vi "UMLEditor SyncCodeFromUml.vi"(7 "Don't Prompt (False)":bool, 8 "error in":errorcluster, 10 "graph":refnum<class "Graph.lvclass">, 11 "selectedNode":refnum<class "AbstractNode.lvclass">) -> (0 "error out":errorcluster)   [LabVIEW 2020]
uses:
  <resource>/Framework/Providers/Open_GDS/UML/AbstractNode_class/AbstractNode.lvclass
  <resource>/Framework/Providers/Open_GDS/UML/Graph_class/Graph.lvclass
  <resource>/Framework/Providers/Open_GDS/UML/ClassNode_class/ExternalSetTypes.ctl
  <resource>/Framework/Providers/Open_GDS/UML/ClassNode_class/ClassNode.lvclass
  C:/Program Files (x86)/National Instruments/LabVIEW 2020/resource/Framework/Providers/Open_GDS/UML/AbstractNode_class/AbstractNode.lvclass
  <resource>/Framework/Providers/Open_GDS/ClassProviders/Common/CommonVIs/CommonVIs_ClassNamePathType.ctl
  <resource>/Framework/Providers/Open_GDS/UML/ClassRelationshipEdge_class/ClassRelationshipEdge.lvclass
  <resource>/Framework/Providers/Open_GDS/UML/AbstractEdge_class/AbstractEdge.lvclass
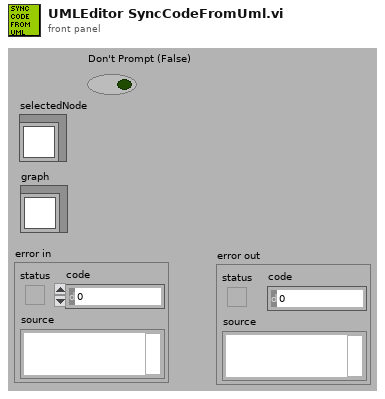
[diagram p1: front panel]
types:
  T1 = typedef "ClassNode.lvclass/ExternalSetTypes.ctl" = enum16{"Name", "Attributes", "Methods", "Position", "ShowMethods", "ShowAttributes", "ClassPath"}
  T2 = typedef "CommonVIs_ClassNamePathType.ctl" = cluster{"ClassNamn":string, "ClassPath":path, "InterfaceClass":bool}
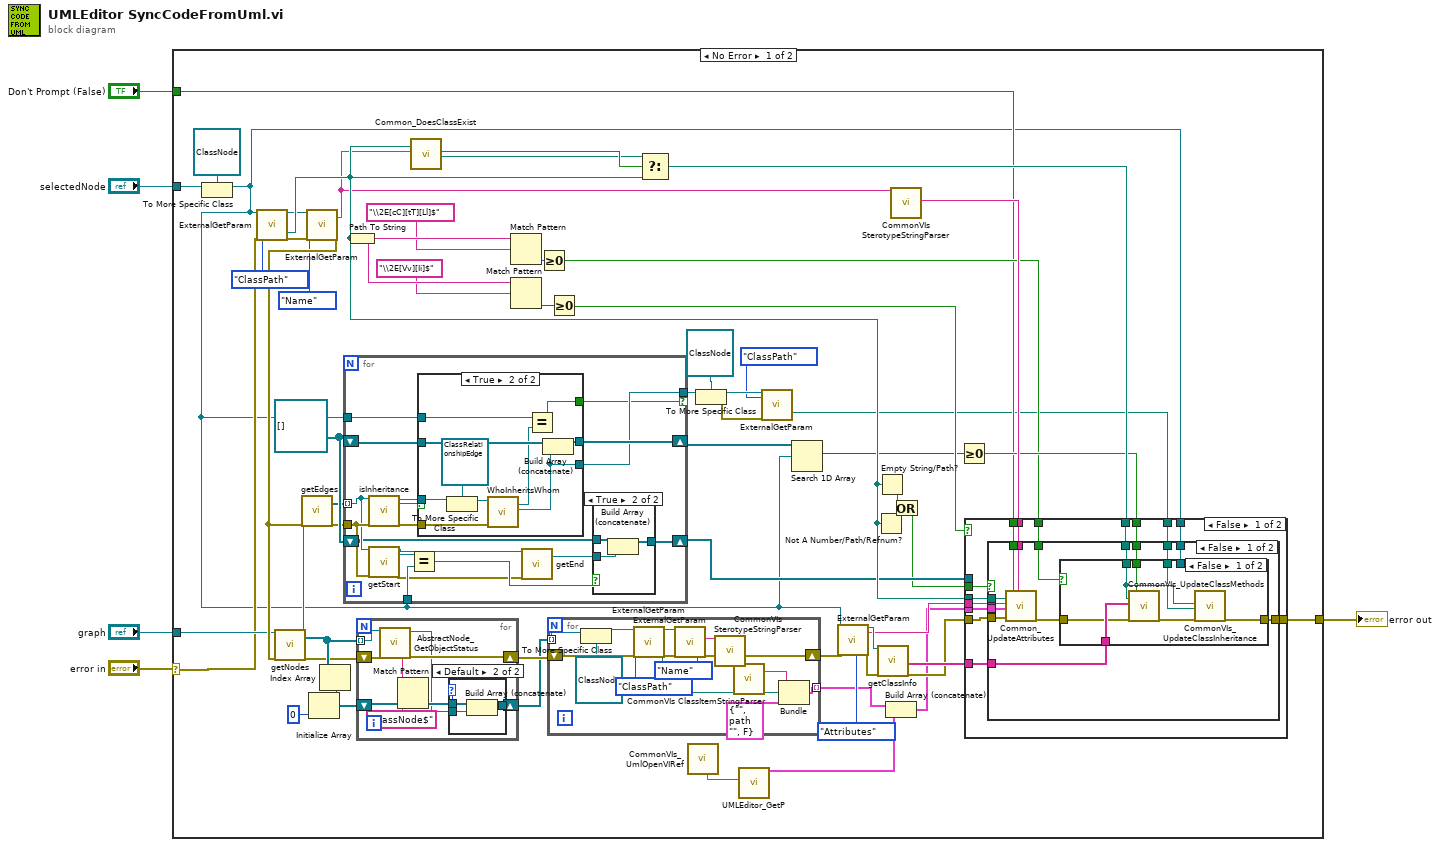
[diagram p0: block diagram]
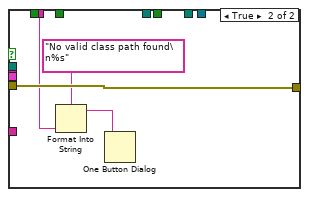
[diagram p3: hidden frame]
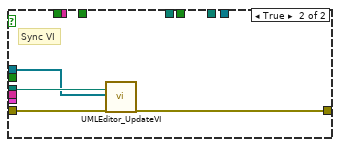
[diagram p4: hidden frame]
diagram:
  n1 = case shown="No Error" "error in" {
    selector: "error in" -> [w13 w171]
    tunnel: [w43 w171] -> w5
    tunnel: "graph" -> [w27 _]
    tunnel: "Don't Prompt (False)" -> [w20 _]
    tunnel: "selectedNode" -> [w14 _]
    frame No Error {
      w63 = refnum<class "AbstractNode.lvclass">[] []
      n2 = To More Specific Class(target class=refnum<class "ClassNode.lvclass"> refnum ("reference"), reference=w14) -> (specific class reference=w12:refnum<class "ClassNode.lvclass">)  [unwired: 1 in, 1 out]
      n3 = call <resource>:"ExternalGetParam.vi"("reference"=w12, "setParameter"=ExternalSetTypes."ClassPath", "error in (no error)"=w13) -> ("reference out"=w44:refnum<class "ClassNode.lvclass">, "Path"=w65:path, "error out"=w45:errorcluster)  [unwired: 14 out]
      n4 = call <resource>:"ExternalGetParam.vi"("reference"=w44, "setParameter"=ExternalSetTypes."Name", "error in (no error)"=w45) -> ("string"=w55:string, "error out"=w47:errorcluster)  [unwired: 15 out]
      n5 = call-dynamic "getNodes.vi"("reference"=w27, "error in (no error)"=w47) -> ("reference out"=w48:refnum<class "Graph.lvclass">, "nodes"=w26:refnum<class "AbstractNode.lvclass">[], "error out"=w25:errorcluster)  [unwired: 15 in]
      n6 = call-dynamic "getEdges.vi"("reference"=w48, "error in (no error)"=w47) -> ("edges"=w50:refnum<class "AbstractEdge.lvclass">[], "error out"=w49:errorcluster)  [unwired: 15 in, 1 out]
      n7 = Index Array(array=w26) -> (element=w22:refnum<class "AbstractNode.lvclass">)  [unwired: 1 in]
      n8 = Initialize Array(w22, 0 ("dimension size")) -> (w24:refnum<class "AbstractNode.lvclass">[])
      n9 = for {
        tunnel: w49 -> [w122]
        tunnel: w50 -> [w121] mode=indexing
        shift-right: [w124] -> w51
        shift-left: w63 -> [w125]
        tunnel: w12 -> [w120]
        shift-right: [w113] -> w64
        shift-left: w63 -> [w115]
        tunnel: w12 -> [w112]
        tunnel: [w111] -> w10 if=w110
        n10 = call-dynamic "isInheritance.vi"("reference"=w121, "error in (no error)"=w122) -> ("reference out"=w123:refnum<class "AbstractEdge.lvclass">, "isInheritance"=w126:bool, "error out"=w127:errorcluster)  [unwired: 13 in, 2 out]
        n11 = call-dynamic "getStart.vi"("reference"=w121, "error in (no error)"=w122) -> ("reference out"=w116:refnum<class "AbstractEdge.lvclass">, "startNode"=w119:refnum<class "AbstractNode.lvclass">, "error out"=w117:errorcluster)  [unwired: 14 in, 1 out]
        n12 = Equal?(x=w119, y=w120) -> (x = y?=w118:bool)
        n13 = case shown="True" w126 {
          tunnel: w127 -> [_ w142]
          tunnel: w125 -> [w132 w141]
          tunnel: [w132 w140] -> w124
          tunnel: w123 -> [_ w139]
          tunnel: w112 -> [_ w136]
          tunnel: [_ w134] -> w111
          tunnel: [_ w133] -> w110
          frame False {
          }
          frame True {
            n14 = To More Specific Class(target class=refnum<class "ClassRelationshipEdge.lvclass"> refnum ("reference"), reference=w139) -> (specific class reference=w137:refnum<class "ClassRelationshipEdge.lvclass">)  [unwired: 1 in, 1 out]
            n15 = call <resource>:"WhoInheritsWhom.vi"("reference"=w137, "error in (no error)"=w142) -> ("inherits"=w135:refnum<class "AbstractNode.lvclass">, "base"=w134:refnum<class "AbstractNode.lvclass">)  [unwired: 16 out]
            n16 = Equal?(x=w136, y=w135) -> (x = y?=w133:bool)
            n17 = Build Array (concatenate)(w141, w134) -> (w140:refnum<class "AbstractNode.lvclass">[])
          }
        }
        n18 = call-dynamic "getEnd.vi"("reference"=w116, "error in (no error)"=w117) -> ("endNode"=w114:refnum<class "AbstractNode.lvclass">)  [unwired: 14 in, 3 out]
        n19 = case shown="True" w118 {
          tunnel: w115 -> [w128 w131]
          tunnel: w114 -> [_ w130]
          tunnel: [w128 w129] -> w113
          frame False {
          }
          frame True {
            n20 = Build Array (concatenate)(w131, w130) -> (w129:refnum<class "AbstractNode.lvclass">[])
          }
        }
      }
      n21 = Path To String(path=w65) -> (string=w61:string)
      n22 = for {
        shift-right: [w164] -> w29
        shift-left: w25 -> [w166]
        tunnel: w26 -> [w165] mode=indexing
        shift-right: [w161] -> w28
        shift-left: w24 -> [w163]
        n23 = call <resource>:"AbstractNode_GetObjectStatus.vi"("reference in"=w165, "error in (no error)"=w166) -> ("Class name"=w160:string, "reference out"=w162:refnum<class "AbstractNode.lvclass">, "error out"=w164:errorcluster)  [unwired: 15 out]
        n24 = Match Pattern(string=w160, regular expression="ClassNode$") -> (offset past match=w158:i32)  [unwired: 4 out]
        n25 = case shown="Default" w158 {
          tunnel: w163 -> [w167 w170]
          tunnel: w162 -> [_ w169]
          tunnel: [w167 w168] -> w161
          frame -1 {
          }
          frame Default {
            n26 = Build Array (concatenate)(w170, w169) -> (w168:refnum<class "AbstractNode.lvclass">[])
          }
        }
      }
      n27 = call <resource>:"Common_DoesClassExist.vi"("ClassPath"=w65, "ClassName"=w55) -> ("llb-class"=w57:bool, "llb/LvCLass-Path"=w56:path)  [unwired: 16 out]
      n28 = Match Pattern(string=w61, regular expression="\\2E[cC][tT][Ll]$") -> (offset past match=w33:i32)  [unwired: 4 out]
      n29 = Match Pattern(string=w61, regular expression="\\2E[Vv][Ii]$") -> (offset past match=w59:i32)  [unwired: 4 out]
      n30 = Greater Or Equal To 0?(x=w33) -> (x >= 0?=w39:bool)
      n31 = for {
        tunnel: w28 -> [w145] mode=indexing
        shift-right: [w152] -> w30
        shift-left: w29 -> [w156]
        tunnel: [w151] -> w16 mode=indexing
        n32 = To More Specific Class(target class=refnum<class "ClassNode.lvclass"> refnum ("reference"), reference=w145) -> (specific class reference=w144:refnum<class "ClassNode.lvclass">)  [unwired: 1 in, 1 out]
        n33 = call <resource>:"ExternalGetParam.vi"("reference"=w144, "setParameter"=ExternalSetTypes."ClassPath", "error in (no error)"=w156) -> ("reference out"=w153:refnum<class "ClassNode.lvclass">, "Path"=w149:path, "error out"=w155:errorcluster)  [unwired: 14 out]
        n34 = call <resource>:"ExternalGetParam.vi"("reference"=w153, "setParameter"=ExternalSetTypes."Name", "error in (no error)"=w155) -> ("string"=w150:string, "error out"=w152:errorcluster)  [unwired: 15 out]
        n35 = call <resource>:"CommonVIs SterotypeStringParser.vi"("SterotypeStringIn"=w150) -> ("Name"=w148:string)  [unwired: 18 out]
        n36 = call <resource>:"CommonVIs ClassItemStringParser.vi"("ClassItemNameIn"=w148) -> ("Name"=w147:string)  [unwired: 18 out]
        n37 = Bundle(cluster=T2 {"ClassNamn"="", "ClassPath"=path "", "InterfaceClass"=FALSE} ("Cluster"), "ClassNamn"=w147, "ClassPath"=w149) -> (w151:T2)  [unwired: 1 in]
      }
      n38 = Greater Or Equal To 0?(x=w59) -> (x >= 0?=w62:bool)
      n39 = Select(t=w56, s=w57, f=w65) -> (s? t:f=w58:path)
      n40 = call <resource>:"CommonVIs_UmlOpenVIRef.vi"() -> ("ProjectNameOut"=w19:string)  [unwired: 4 in, 7 out]
      n41 = To More Specific Class(target class=refnum<class "ClassNode.lvclass"> refnum ("reference"), reference=w10) -> (specific class reference=w9:refnum<class "ClassNode.lvclass">, error out=w8:errorcluster)  [unwired: 1 in]
      n42 = call <resource>:"UMLEditor_GetP.vi"("GetProjectRefByName/or Ref"=w19) -> ("ClassesNamesAndPaths"=w18:T2[])  [unwired: 1 in, 9 out]
      n43 = call <resource>:"ExternalGetParam.vi"("reference"=w9, "setParameter"=ExternalSetTypes."ClassPath", "error in (no error)"=w8) -> ("Path"=w6:path)  [unwired: 16 out]
      n44 = Search 1D Array(1D array=w51, element=w12) -> (index of element=w52:i32)  [unwired: 1 out]
      n45 = call <resource>:"ExternalGetParam.vi"("reference"=w12, "setParameter"=ExternalSetTypes."Attributes", "error in (no error)"=w30) -> ("reference out"=w41:refnum<class "ClassNode.lvclass">, "string"=w40:string, "error out"=w42:errorcluster)  [unwired: 14 out]
      n46 = Not A Number/Path/Refnum?(number/path/refnum=w65) -> (NaN/Path/Refnum?=w35:bool)
      n47 = Empty String/Path?(string/path=w65) -> (empty?=w34:bool)
      n48 = call-dynamic "getClassInfo.vi"("reference"=w41, "error in (no error)"=w42) -> ("methods"=w38:string[], "error out"=w37:errorcluster)  [unwired: 8 in, 8 out]
      n49 = Build Array (concatenate)(w16, w18) -> (w17:T2[])
      n50 = call <resource>:"CommonVIs SterotypeStringParser.vi"("SterotypeStringIn"=w55) -> ("Sterotype"=w54:string)  [unwired: 18 out]
      n51 = Or(x=w34, y=w35) -> (x .or. y?=w36:bool)
      n52 = Greater Or Equal To 0?(x=w52) -> (x >= 0?=w53:bool)
      n53 = case shown="False" w62 {
        tunnel: w36 -> [w79 _]
        tunnel: w37 -> [w78 w109]
        tunnel: w38 -> [w77 _]
        tunnel: w65 -> [w76 w107]
        tunnel: w39 -> [w75 _]
        tunnel: w17 -> [w74 _]
        tunnel: w40 -> [w73 _]
        tunnel: [w72 w108] -> w43
        tunnel: w53 -> [w71 _]
        tunnel: w54 -> [w70 _]
        tunnel: w58 -> [w69 _]
        tunnel: w64 -> [_ w106]
        tunnel: w20 -> [w68 _]
        tunnel: w12 -> [w67 _]
        tunnel: w6 -> [w66 _]
        frame False {
          n54 = case shown="False" w79 {
            tunnel: [w88 w105] -> w72
            tunnel: w73 -> [w93 _]
            tunnel: w78 -> [w92 w105]
            tunnel: w74 -> [w91 _]
            tunnel: w76 -> [w90 _]
            tunnel: w75 -> [w87 _]
            tunnel: w69 -> [w86 _]
            tunnel: w77 -> [w85 _]
            tunnel: w71 -> [w84 _]
            tunnel: w70 -> [w83 w102]
            tunnel: w68 -> [w82 _]
            tunnel: w67 -> [w81 _]
            tunnel: w66 -> [w80 _]
            frame False {
              n55 = call <resource>:"Common_UpdateAttributes.vi"("ClassPath/LvClassRef"=w90, "NewAttributes"=w93, "ClassInfo"=w91, "error in (no error)"=w92, "Don't Prompt (False)"=w82, "Stereotype"=w83) -> ("error out"=w89:errorcluster)  [unwired: 13 out]
              n56 = case shown="False" w87 {
                tunnel: w89 -> [w98 w101]
                tunnel: [w97 w101] -> w88
                tunnel: w86 -> [w96 _]
                tunnel: w85 -> [w99 _]
                tunnel: w84 -> [w95 _]
                tunnel: w81 -> [_ _]
                tunnel: w80 -> [w94 _]
                frame False {
                  n57 = call <resource>:"CommonVIs_UpdateClassMethods.vi"("ClassPath/LvClassRef"=w96, "Methods"=w99, "error in (no error)"=w98, "BaseClass"=w95) -> ("error out"=w100:errorcluster)  [unwired: 3 in, 12 out]
                  n58 = call <resource>:"CommonVIs_UpdateClassInheritance.vi"("ClassPath/LvClassRef"=w96, "ParentClass"=w94, "error in (no error)"=w100) -> ("error out"=w97:errorcluster)  [unwired: 16 in]
                }
                frame True {
                }
              }
            }
            frame True {
              n59 = Format Into String(format string="No valid class path found\n%s" ("message"), w102) -> (resulting string=w103:string)  [unwired: 2 in, 1 out]
              n60 = One Button Dialog(message=w103) -> ()  [unwired: 2 out]
            }
          }
        }
        frame True {
          # "Sync VI"
          n61 = call <resource>:"UMLEditor_UpdateVI.vi"("ViPath"=w107, "DependendClasses"=w106, "error in (no error)"=w109) -> ("error out"=w108:errorcluster)  [unwired: 16 out]
        }
      }
    }
    frame Error {
    }
  }
  "error out" <- w5
